vi "test Counter-Driven Output.vi"(8 "error in (no error)":errorcluster, 11 "TestCase in":refnum<class "Scan Engine Specialty Digital System Tests.lvclass">) -> (0 "error out":errorcluster, 3 "TestCase out":refnum<class "Scan Engine Specialty Digital System Tests.lvclass">)   [LabVIEW 2020, in "Scan Engine Specialty Digital System Tests.lvclass"]
uses:
  Scan Engine Specialty Digital System Tests.lvclass
  C:/Program Files (x86)/National Instruments/LabVIEW 2020/vi.lib/NI/VeriStand Custom Device Testing Tools/VeriStandTestCase/VeriStandTestCase.lvclass
  <vilib>/addons/_JKI Toolkits/VI Tester/TestCase.llb/TestCase.lvclass
  <vilib>/NI/VeriStand Custom Device Testing Tools/VeriStandTestUtilities/VeriStandTestUtilities.lvlib
  C:/Program Files (x86)/National Instruments/LabVIEW 2020/vi.lib/addons/_JKI Toolkits/VI Tester/TestCase.llb/TestCase.lvclass
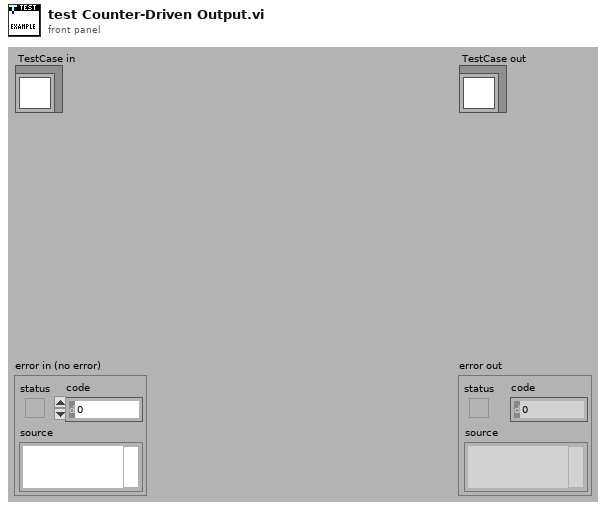
[diagram p1: front panel]
types:
  T1 = typedef "NI_VS Workspace ExecutionAPI.lvlib/WorkspaceAPI.ctl" = refnum<k24>
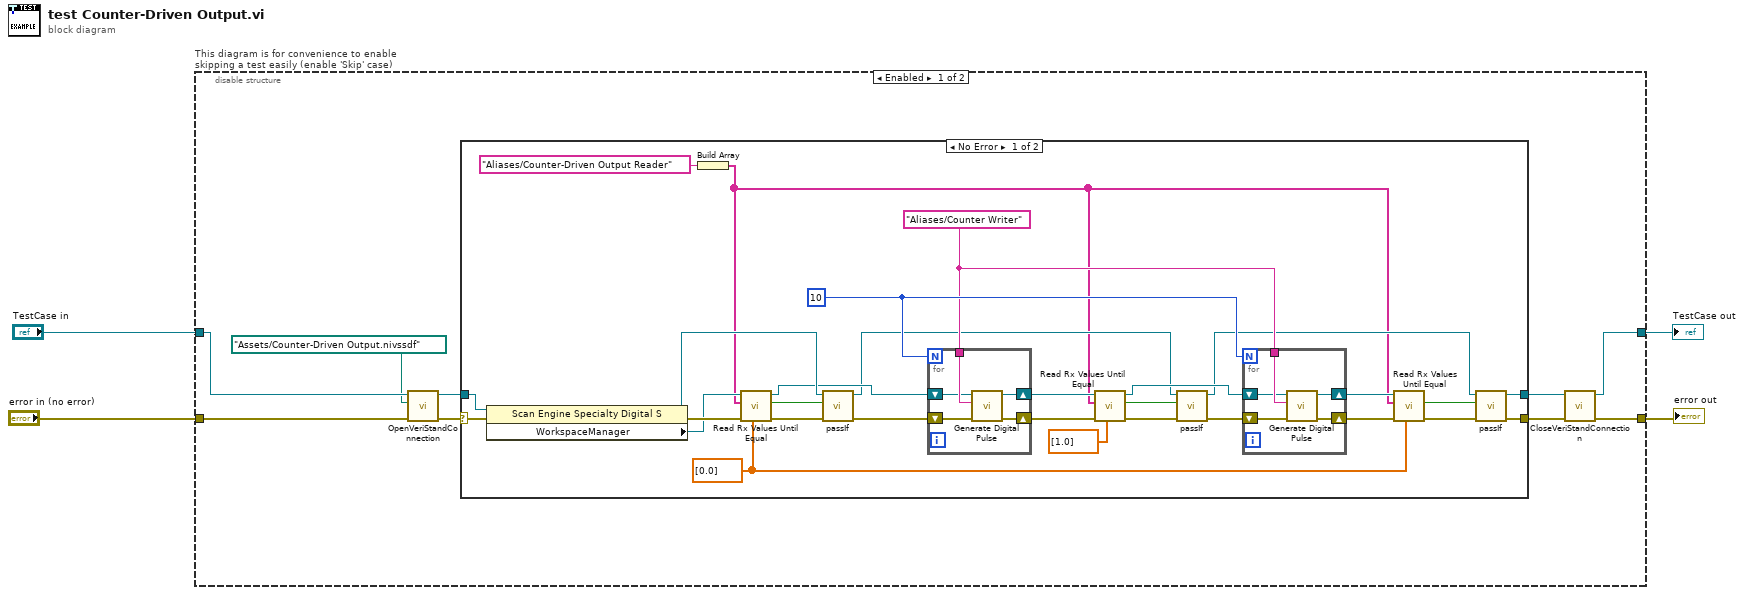
[diagram p0: block diagram]
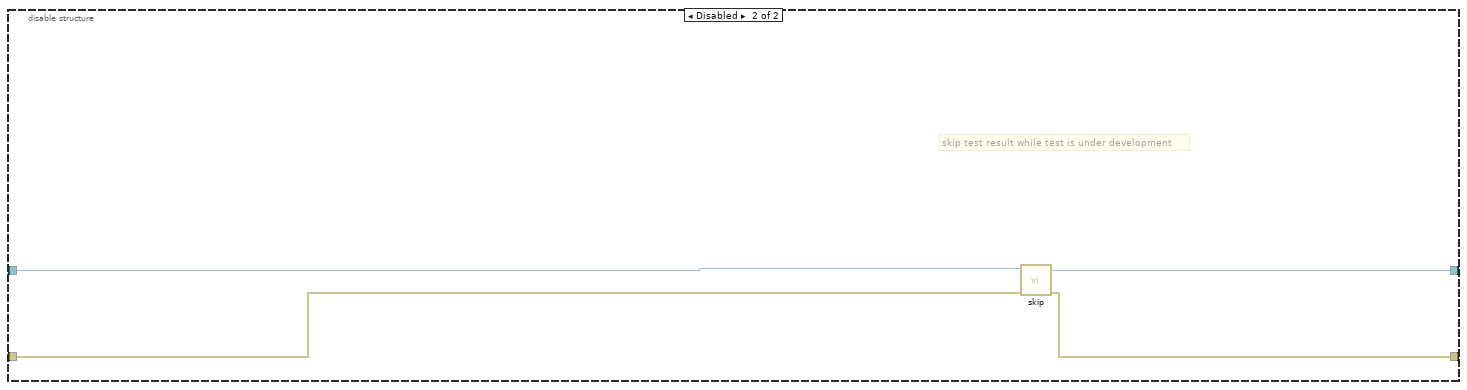
[diagram p3: hidden frame]
diagram:
  n1 = disable-structure "This diagram is for convenience to enable skipping a test easily (enable 'Skip' case)" shown="Enabled" {
    disable-tunnel: "TestCase in" -> [w13 w58]
    disable-tunnel: [w8 w56] -> w1
    disable-tunnel: [w6 w57] -> w3
    disable-tunnel: "error in (no error)" -> [w10 w55]
    frame Enabled {
      n2 = call-dynamic "OpenVeriStandConnection.vi"("error in (no error)"=w10, "System Definition File"=path "Assets/Counter-Driven Output.nivssdf", "VeriStand Test Case in"=w13) -> ("error out"=w11:errorcluster, "VeriStand Test Case out"=w12:refnum<class "Scan Engine Specialty Digital System Tests.lvclass">)  [unwired: 6 in, 1 out]
      n3 = case shown="No Error" w11 {
        selector: w11 -> [w22 w53]
        tunnel: w12 -> [w23 w54]
        tunnel: [w21 w54] -> w9
        tunnel: [w20 w53] -> w7
        frame No Error {
          w14 = dbl[] [0.0]
          w36 = 10 ("Terminal Count")
          w35 = "Aliases/Counter Writer" ("Channel")
          n4 = property class="Scan Engine Specialty Digital S"(reference=w23, error in=w22) -> (reference out=w41:refnum<class "Scan Engine Specialty Digital System Tests.lvclass">, error out=w40:errorcluster, "WorkspaceManager"=w38:T1)
          n5 = Build Array("Aliases/Counter-Driven Output Reader" ("Channel")) -> (w19:string[])
          n6 = call <vilib>:"Read Rx Values Until Equal.vi"("expected values"=w14, "error in"=w40, "Rx aliases"=w19, "workspace manager in"=w38) -> ("error out"=w39:errorcluster, "values equal expected"=w18:bool, "workspace manager out"=w37:T1)  [unwired: 5 in]
          n7 = call-dynamic "passIf.vi"("error in (no error)"=w39, "pass"=w18, "TestCase in"=w41) -> ("error out"=w42:errorcluster, "TestCase out"=w29:refnum<class "Scan Engine Specialty Digital System Tests.lvclass">)  [unwired: 7 in]
          n8 = for {
            N: w36 -> [_]
            shift-right: [w51] -> w32
            shift-left: w42 -> [w52]
            tunnel: w35 -> [w50]
            shift-right: [w48] -> w31
            shift-left: w37 -> [w49]
            n9 = call "Generate Digital Pulse.vi"("error in (no error)"=w52, "Channel"=w50, "WorkspaceManager"=w49) -> ("error out"=w51:errorcluster, "Workspace Manager out"=w48:T1)  [unwired: 7 in]
          }
          n10 = call <vilib>:"Read Rx Values Until Equal.vi"("expected values"=dbl[] [1.0], "error in"=w32, "Rx aliases"=w19, "workspace manager in"=w31) -> ("error out"=w34:errorcluster, "values equal expected"=w16:bool, "workspace manager out"=w30:T1)  [unwired: 5 in]
          n11 = call-dynamic "passIf.vi"("error in (no error)"=w34, "pass"=w16, "TestCase in"=w29) -> ("error out"=w33:errorcluster, "TestCase out"=w26:refnum<class "Scan Engine Specialty Digital System Tests.lvclass">)  [unwired: 7 in]
          n12 = for {
            N: w36 -> [_]
            shift-right: [w46] -> w27
            shift-left: w33 -> [w47]
            tunnel: w35 -> [w45]
            shift-right: [w43] -> w25
            shift-left: w30 -> [w44]
            n13 = call "Generate Digital Pulse.vi"("error in (no error)"=w47, "Channel"=w45, "WorkspaceManager"=w44) -> ("error out"=w46:errorcluster, "Workspace Manager out"=w43:T1)  [unwired: 7 in]
          }
          n14 = call <vilib>:"Read Rx Values Until Equal.vi"("expected values"=w14, "error in"=w27, "Rx aliases"=w19, "workspace manager in"=w25) -> ("error out"=w28:errorcluster, "values equal expected"=w15:bool)  [unwired: 5 in, 1 out]
          n15 = call-dynamic "passIf.vi"("error in (no error)"=w28, "pass"=w15, "TestCase in"=w26) -> ("error out"=w20:errorcluster, "TestCase out"=w21:refnum<class "Scan Engine Specialty Digital System Tests.lvclass">)  [unwired: 7 in]
        }
        frame Error {
        }
      }
      n16 = call-dynamic "CloseVeriStandConnection.vi"("error in (no error)"=w7, "VeriStand Test Case in"=w9) -> ("error out"=w6:errorcluster, "VeriStand Test Case out"=w8:refnum<class "Scan Engine Specialty Digital System Tests.lvclass">)  [unwired: 8 in]
    }
    frame Disabled {
      # "skip test result while test is under development"
      n17 = call <vilib>:"skip.vi"("error in (no error)"=w55, "TestCase in"=w58) -> ("error out"=w57:errorcluster, "TestCase out"=w56:refnum<class "Scan Engine Specialty Digital System Tests.lvclass">)  [unwired: 8 in]
    }
  }
  "error out" <- w3
  "TestCase out" <- w1
